vi "CreatePublicEvents.vi"(8 "error in (no error)":errorcluster, 11 "Microscope":refnum<class "Microscope.lvclass">) -> (0 "error out":errorcluster, 3 "Microscope out":refnum<class "Microscope.lvclass">)   [LabVIEW 2013, in "Microscope.lvclass"]
doc: "---------------------------------------------------------------\nJKI State Machine Objects™\nhttp://jki.net/state-machine-objects/\nCopyright (C) 2005-2015, JKI <info@jki.net>\nALL RIGHTS RESERVEDJKI State Machine Objects (SMO) 1.0.0.5\nJKI - JKI\nCopyright (c) 2016, JKI"
uses:
  Microscope.lvclass
  Typedefs/ValueChanged--EventData--Cluster.ctl
  <vilib>/JKI/JKI SMO/SMO/SMO.lvclass
  Typedefs/PublicEvents--Microscope.Initialized.ctl
panel:
  # "For instructions on how to use the JKI State Machine Objects, examples and video tutorials, visit:\nhttp://jki.net/state-machine-objects/\n\nJKI State Machine Objects™\nhttp://jki.net/state-machine-objects/\nCopyright (C) 2005-2015, JKI <info@jki.net>\nALL RIGHTS RESERVED"
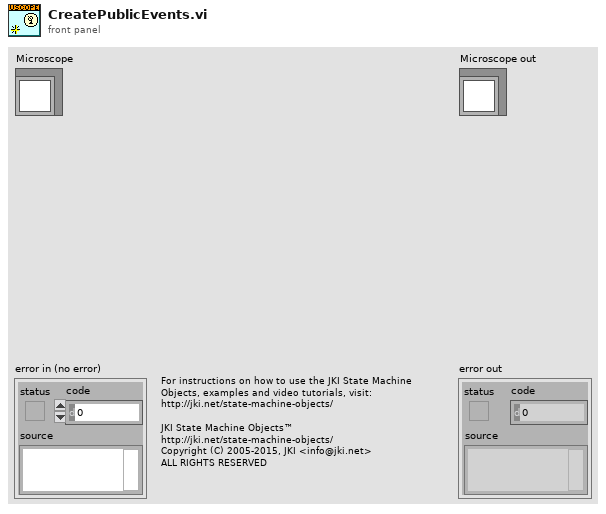
[diagram p1: front panel]
types:
  T1 = typedef "Microscope.lvclass/ValueChanged--EventData--Cluster.ctl" = cluster{"New Value":string}
  T2 = typedef "Microscope.lvclass/PrivateData--Ref.ctl" = refnum<data-value>
  T3 = typedef "Microscope.lvclass/PublicEvents--Microscope.Initialized.ctl" = bool
  T4 = typedef "Microscope.lvclass/PrivateData--Cluster.ctl" = cluster{"Public Events":T5, "Protected Events":T6, "Private Events":T7, "Dependencies":T8, "Configuration":T9}
  T5 = typedef "Microscope.lvclass/PublicEvents--Cluster.ctl" = cluster{"Value Changed":refnum<user-event>, "Initialized":refnum<user-event>}
  T6 = typedef "Microscope.lvclass/ProtectedEvents--Cluster.ctl" = cluster{"placeholder":refnum<user-event>}
  T7 = typedef "Microscope.lvclass/PrivateEvents--Cluster.ctl" = cluster{"New Value":refnum<user-event>, "Initialize":refnum<user-event>, "CaptureImageAtPosition":refnum<user-event>}
  T8 = typedef "Microscope.lvclass/Dependencies--Cluster.ctl" = cluster{"XYStage":refnum<class "XYStage.lvclass">, "Camera":refnum<class "Camera.lvclass">}
  T9 = typedef "Microscope.lvclass/Configuration--Cluster.ctl" = cluster{"XY Stage":string, "Camera":string, "image output folder":path, "filetype":string}
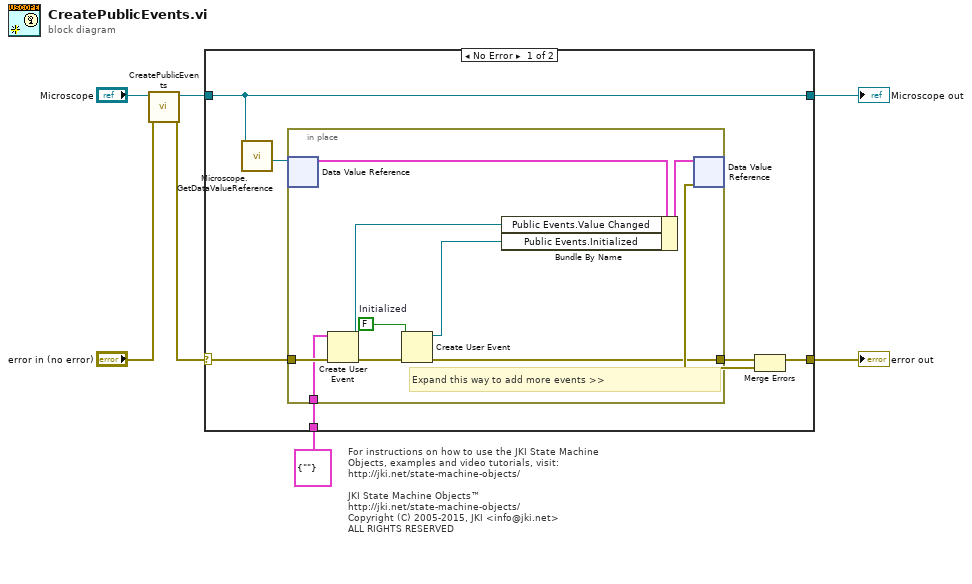
[diagram p0: block diagram]
diagram:
  # "For instructions on how to use the JKI State Machine Objects, examples and video tutorials, visit:\nhttp://jki.net/state-machine-objects/\n\nJKI State Machine Objects™\nhttp://jki.net/state-machine-objects/\nCopyright (C) 2005-2015, JKI <info@jki.net>\nALL RIGHTS RESERVED"
  n1 = call-parent "CreatePublicEvents.vi"("error in (no error)"="error in (no error)", "SMO"="Microscope") -> ("error out"=w1:errorcluster, "SMO out"=w3:refnum<class "Microscope.lvclass">)  [unwired: 8 in]
  n2 = case shown="No Error" w1 {
    selector: w1 -> [w14 w25]
    tunnel: [w13 w25] -> w6
    tunnel: [w9 w24] -> w7
    tunnel: w3 -> [w9 w24]
    tunnel: T1 {"New Value"=""} ("Data In Event Data") -> [w12 _]
    frame No Error {
      n3 = call "Microscope.GetDataValueReference.vi"("Microscope"=w9) -> ("Ref"=w8:T2)  [unwired: 10 in]
      n4 = in-place {
        in-place-border: w14 -> [w20]
        in-place-border: [w17] -> w11
        in-place-border: w12 -> [w19]
        w16 = T3 FALSE  # Initialized
        # "Expand this way to add more events >>"
        n5 = in-place-dvr #1(w8) -> (w22:T4)  [unwired: 1 out]
        n6 = Create User Event(user event datatype=w19, error in=w20) -> (user event=w18:refnum<user-event>, error out=w21:errorcluster)
        n7 = Create User Event(user event datatype=w16, error in=w21) -> (user event=w15:refnum<user-event>, error out=w17:errorcluster)
        n8 = Bundle By Name(cluster=w22, "Public Events.Value Changed"=w18, "Public Events.Initialized"=w15) -> (w23:T4)
        n9 = in-place-dvr #1(w23) -> (w10:errorcluster)  [unwired: 1 out]
      }
      n10 = Merge Errors(w11, w10) -> (w13:errorcluster)
    }
    frame Error {
    }
  }
  "error out" <- w6
  "Microscope out" <- w7
